vi "update run end time.vi"(7 "set to now":bool, 10 "End Time":timestamp format="%<%x %.3X>T", 11 "run":refnum<class "Run.lvclass">) -> (0 "error out":errorcluster, 3 "updated run":refnum<class "Run.lvclass">)   [LabVIEW 2020, in "nominal core steps.lvlib"]
doc: "Change the end time of a run."
uses:
  nominal core steps.lvlib
  <vilib>/Nominal/Nominal IO Client/lv_src/Run/Run.lvclass
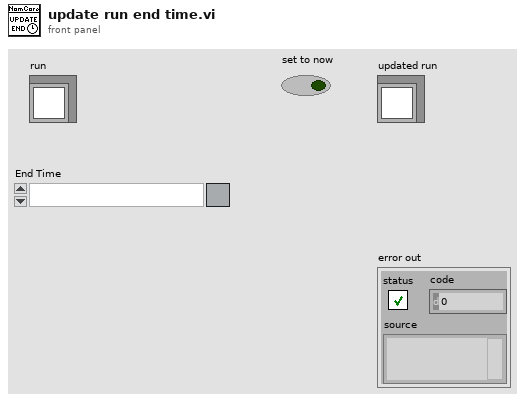
[diagram p1: front panel]
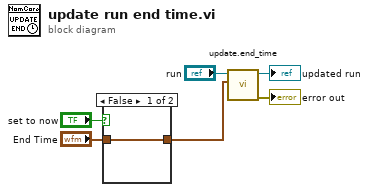
[diagram p0: block diagram]
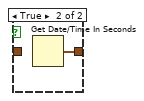
[diagram p2: hidden frame]
diagram:
  n1 = case shown="False" "set to now" {
    tunnel: [w7 w8] -> w2
    tunnel: "End Time" -> [w7 _]
    frame False {
    }
    frame True {
      n2 = Get Date/Time In Seconds() -> (seconds since 1Jan1904=w8:timestamp)
    }
  }
  n3 = call <vilib>:"update.end_time.vi"("End Time (now)"=w2, "Run in"="run") -> ("error out"=→"error out":errorcluster, "Run out"=→"updated run":refnum<class "Run.lvclass">)  [unwired: 8 in]
